vi "lvmcp_setpos.vi"() -> ()   [LabVIEW 2015]
panel:
  out "error out":errorcluster
  in  "position":cluster{"Left":i32, "Top":i32}
  in  "reference":refnum<vi>
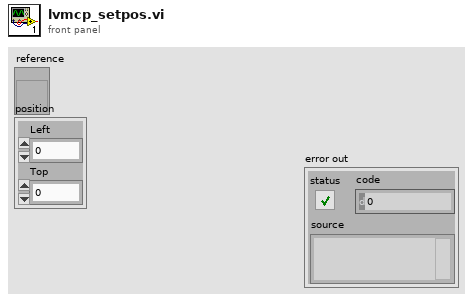
[diagram p1: front panel]
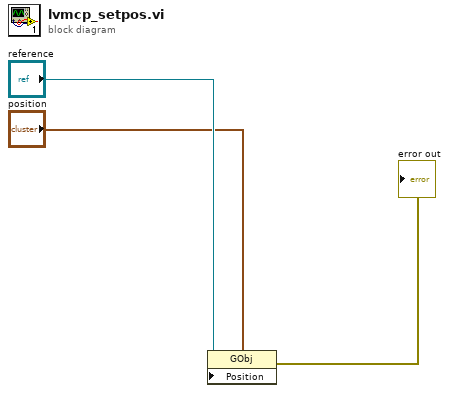
[diagram p0: block diagram]
diagram:
  n1 = property class="GObj"(reference="reference", "Position"="position") -> (error out=→"error out":errorcluster)  [unwired: 1 in, 1 out]
